vi "Get Devices.vi"(6 "timeout (ms)":i32=5000, 8 "error in":errorcluster, 10 "Refresh Device List":bool, 11 "gRPC ID":T2) -> (0 "error out":errorcluster, 2 "devices":T1[](array[typedef]), 3 "gRPC ID out":T2)   [LabVIEW 2021, in "CAN_Reader_NIXNET_Wrapper.lvlib"]
uses:
  CAN_Reader_NIXNET_Wrapper.lvlib
  <vilib>/gRPC/LabVIEW gRPC Library/Shared/grpcId.ctl
  CanReaderNixnet_client/CanReaderNixnet_client.lvlib
  CanReaderNixnet_client/RPC Messages/cif_can_reader_nixnet_RefreshDevices.ctl
  <vilib>/gRPC/LabVIEW gRPC Library/grpc-lvsupport-release.lvlib
  CanReaderNixnet_client/RPC Messages/cif_can_reader_nixnet_XnetDevice.ctl
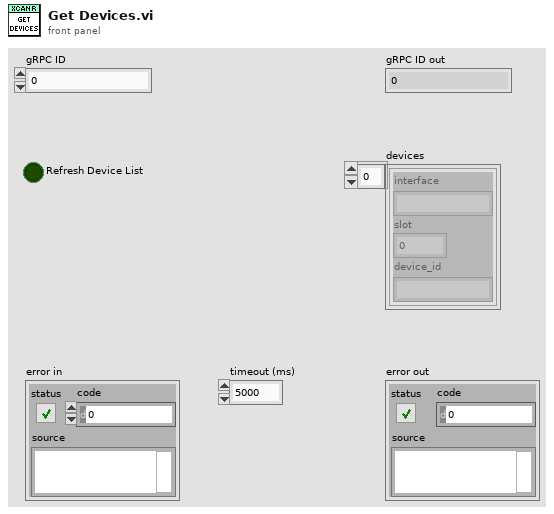
[diagram p1: front panel]
types:
  T1 = typedef "CanReaderNixnet_client.lvlib/cif_can_reader_nixnet_XnetDevice.ctl" = cluster{"interface":string, "slot":u32, "device_id":string}
  T2 = typedef "grpc-lvsupport-release.lvlib/grpcId.ctl" = u64
  T3 = typedef "CanReaderNixnet_client.lvlib/cif_can_reader_nixnet_RefreshDevices.ctl" = cluster{"refresh_device_list":bool}
  T4 = typedef "CanReaderNixnet_client.lvlib/cif_can_reader_nixnet_XnetDevices.ctl" = cluster{"devices":T1[]}
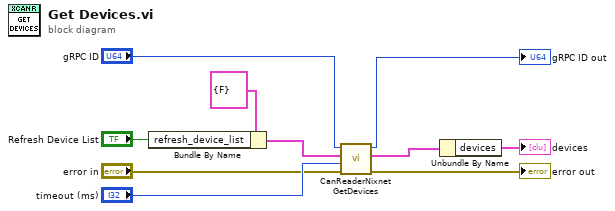
[diagram p0: block diagram]
diagram:
  n1 = Bundle By Name(cluster=T3 {"refresh_device_list"=FALSE} ("Request Data"), "refresh_device_list"="Refresh Device List") -> (w1:T3)
  n2 = call "CanReaderNixnet GetDevices.vi"("error in"="error in", "timeout (ms)"="timeout (ms)", "Request Data"=w1, "gRPC ID"="gRPC ID") -> ("error out"=→"error out":errorcluster, "Response Data"=w5:T4, "gRPC ID out"=→"gRPC ID out":T2)  [unwired: 5 in]
  n3 = Unbundle By Name(w5) -> ("devices"=→"devices":T1[])
